vi "Confocal.vi"() -> ()   [LabVIEW 2024]
panel:
  out "appended array":dbl[](array[numeric])
  in  "N per point":i32=1
  in  "Z Steps?":i32
  out "Intensity Graph":dbl[][](graph)
  in  "Direction":bool
  in  "file path (use dialog) 2":path=path "C:/Users/Crawford Group/Desktop/Angelo/NMR/DATA/Unaveraged&TimeStamp.txt"
  in  "file path (use dialog)":path=path "C:/Users/Crawford Group/Desktop/Angelo/NMR/DATA/DATA.txt"
  out "error out":errorcluster
  in  "Step size mm  Y":dbl=0.0017
  in  "Y Motor":refnum<k7>(container)
  out "error out 2":errorcluster
  in  "Step size mm X":dbl=0.0098
  in  "X Motor":refnum<k7>(container)
  in  "Sweeps (X,Y)":i32=1
  in  "Up?":bool
  in  "Number of X steps":dbl=1.0
  out "Number of X":i32
  out "Y Steps":i32
  out "Direction Indicator":bool
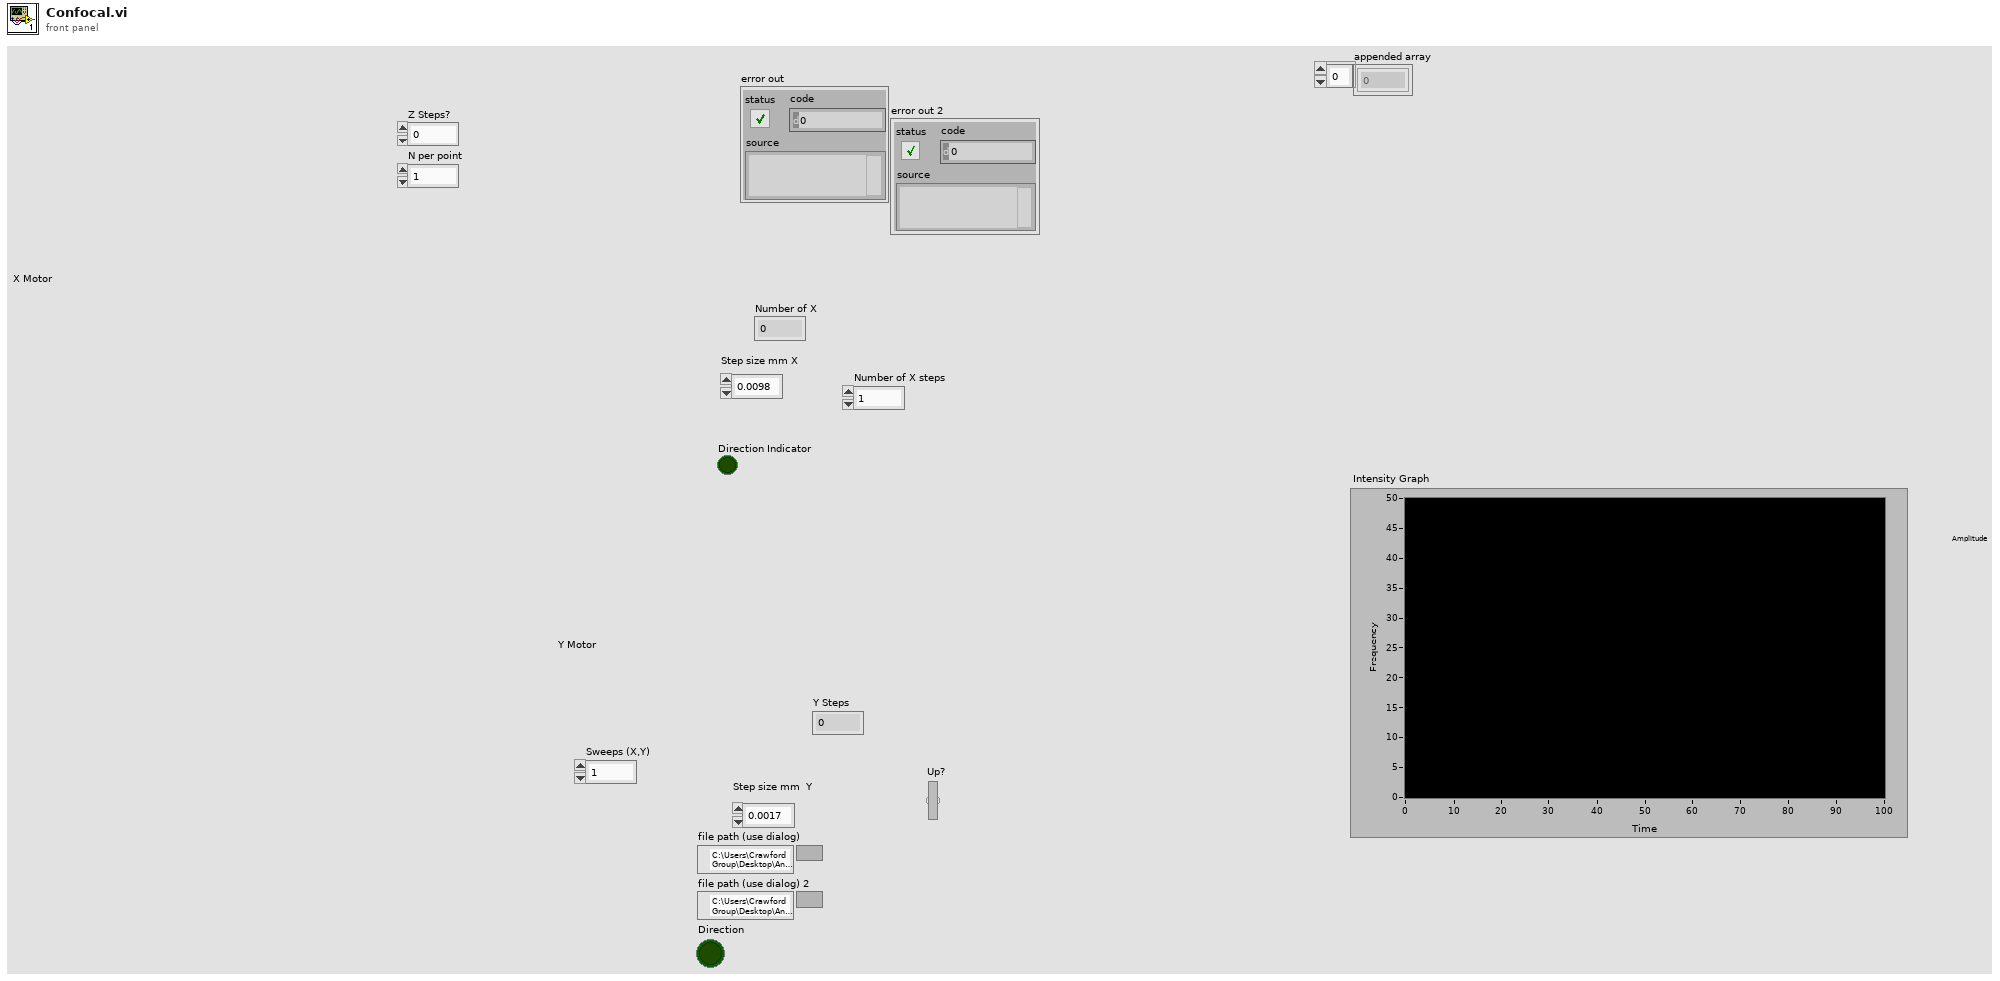
[diagram p1: front panel]
types:
  T1 = enum16{"open", "replace", "create", "open or create", "replace or create", "replace or create with confirmation"}
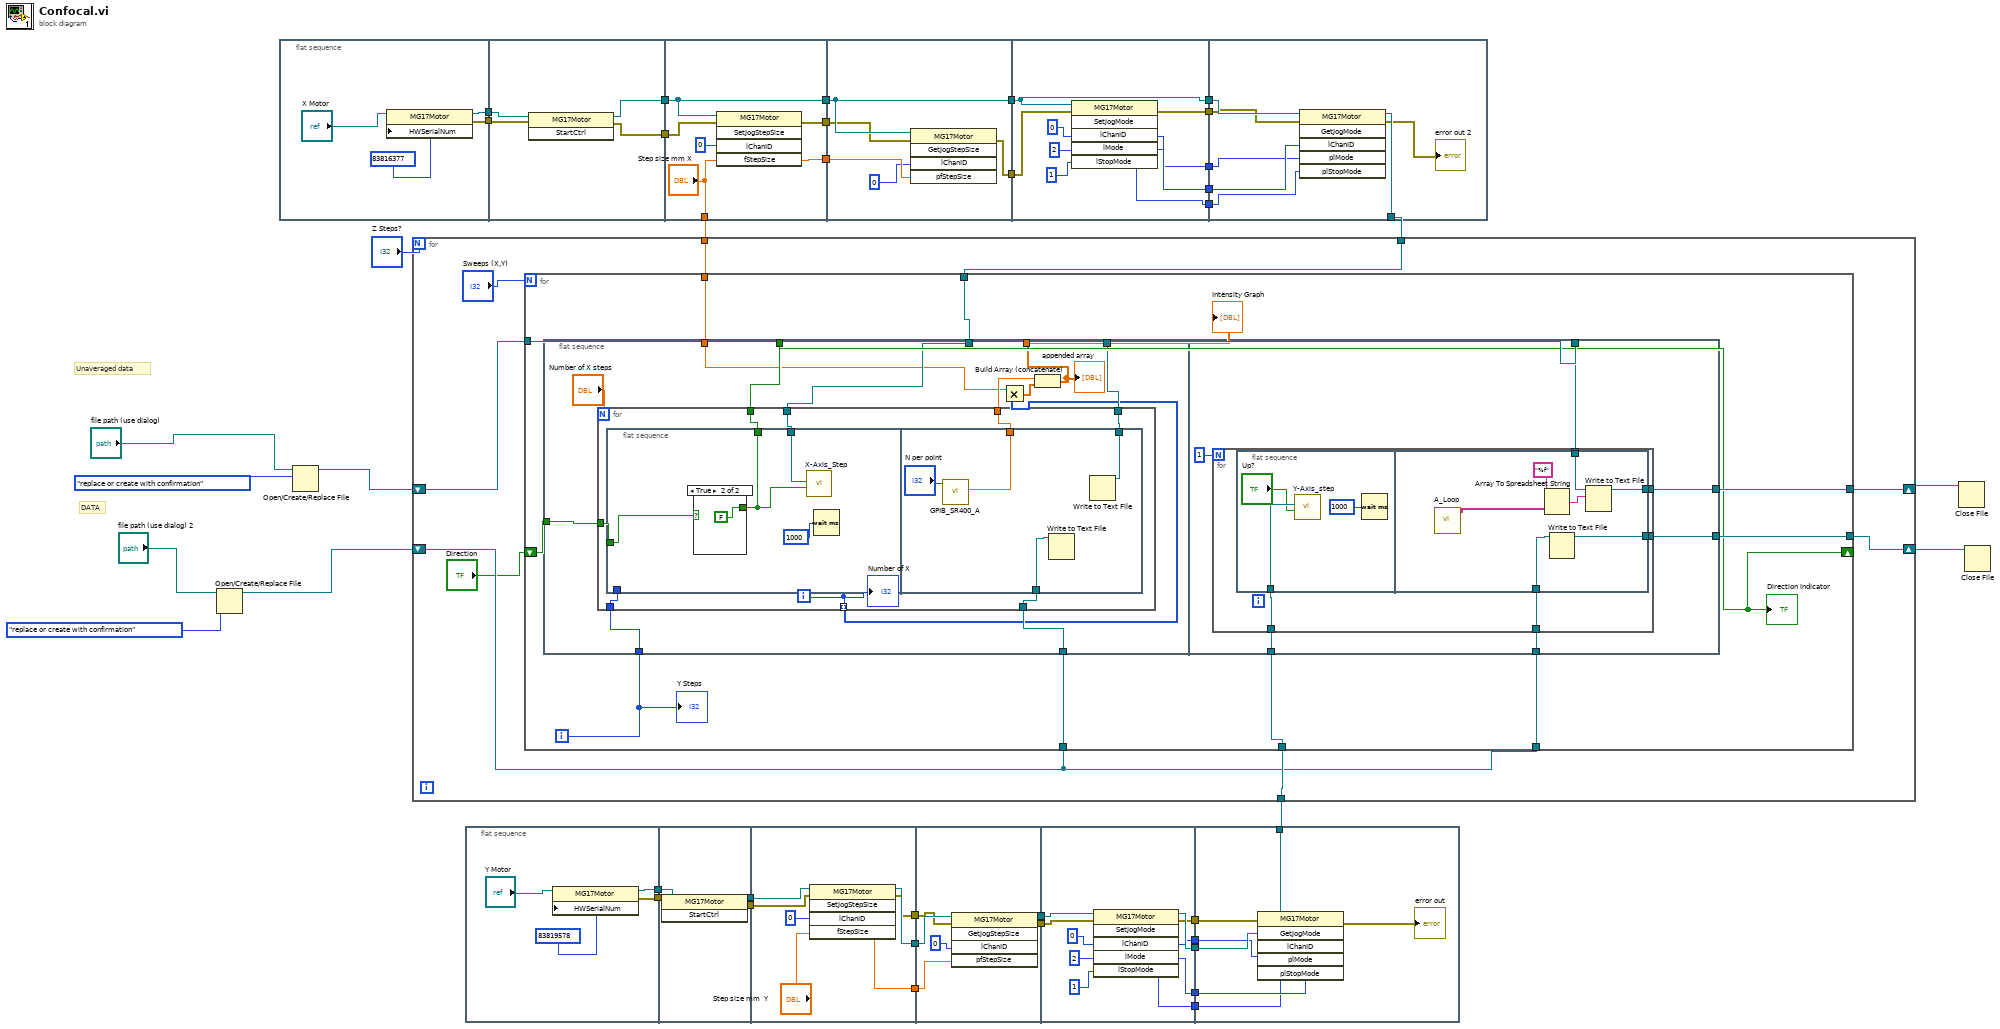
[diagram p0: block diagram]
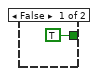
[diagram p2: hidden frame]
diagram:
  # "Unaveraged data"
  # "DATA"
  n1 = Open/Create/Replace File(file path (use dialog)="file path (use dialog) 2", operation (0:open)=T1."replace or create with confirmation") -> (refnum out=w3:refnum<file>)  [unwired: 4 in, 2 out]
  n2 = flat-sequence {
    tunnel: [w42] -> w40
    tunnel: [w41] -> w39
    tunnel: w40 -> [w48]
    tunnel: w39 -> [w47]
    tunnel: [w46] -> w38
    tunnel: [w45] -> w37
    tunnel: w38 -> [w54]
    tunnel: w37 -> [w53]
    tunnel: [w54] -> w36
    tunnel: [w52] -> w35
    tunnel: [w51] -> w34
    tunnel: ["Step size mm X"] -> w1
    tunnel: w36 -> [w59]
    tunnel: w35 -> [w58]
    tunnel: w34 -> [w57]
    tunnel: [w59] -> w33
    tunnel: [w56] -> w32
    tunnel: w33 -> [w68]
    tunnel: w32 -> [w67]
    tunnel: [w68] -> w31
    tunnel: [w63] -> w30
    tunnel: [w62] -> w29
    tunnel: [w61] -> w28
    tunnel: [w60] -> w27
    tunnel: w31 -> [w75]
    tunnel: w30 -> [w74]
    tunnel: w29 -> [w73]
    tunnel: w28 -> [w72]
    tunnel: [w71] -> w12
    tunnel: w27 -> [w69]
    frame #0 {
      n3 = property class="MG17Motor"(reference="X Motor", "HWSerialNum"=83816377) -> (reference out=w42:refnum<k7>, error out=w41:errorcluster)  [unwired: 1 in]
    }
    frame #1 {
      n4 = invoke class="MG17Motor" method="StartCtrl"(reference=w48, error in=w47) -> (reference out=w46:refnum<k7>, error out=w45:errorcluster)  [unwired: 1 in, 1 out]
    }
    frame #2 {
      n5 = invoke class="MG17Motor" method="SetJogStepSize"(reference=w54, error in=w53, "lChanID"=0, "fStepSize"="Step size mm X") -> (error out=w52:errorcluster, "fStepSize"=w51:sgl)  [unwired: 1 in, 3 out]
    }
    frame #3 {
      n6 = invoke class="MG17Motor" method="GetJogStepSize"(reference=w59, error in=w58, "lChanID"=0, "pfStepSize"=w57) -> (error out=w56:errorcluster)  [unwired: 1 in, 4 out]
    }
    frame #4 {
      n7 = invoke class="MG17Motor" method="SetJogMode"(reference=w68, error in=w67, "lChanID"=0, "lMode"=2, "lStopMode"=1) -> (error out=w63:errorcluster, "lChanID"=w62:i32, "lMode"=w61:i32, "lStopMode"=w60:i32)  [unwired: 1 in, 2 out]
    }
    frame #5 {
      n8 = invoke class="MG17Motor" method="GetJogMode"(reference=w75, error in=w74, "lChanID"=w73, "plMode"=w72, "plStopMode"=w69) -> (reference out=w71:refnum<k7>, error out=→"error out 2":errorcluster)  [unwired: 1 in, 4 out]
    }
  }
  n9 = Open/Create/Replace File(file path (use dialog)="file path (use dialog)", operation (0:open)=T1."replace or create with confirmation") -> (refnum out=w5:refnum<file>)  [unwired: 4 in, 2 out]
  n10 = for {
    N: "Z Steps?" -> [_]
    tunnel: w12 -> [w83]
    tunnel: w11 -> [w82]
    shift-right: [w81] -> w6
    shift-left: w5 -> [w80]
    shift-right: [w79] -> w4
    shift-left: w3 -> [w78]
    tunnel: w1 -> [w76]
    n11 = for {
      N: "Sweeps (X,Y)" -> [_]
      tunnel: w82 -> [w96]
      tunnel: w83 -> [w95]
      tunnel: [w94] -> w81
      tunnel: w80 -> [w91]
      tunnel: w78 -> [w93]
      tunnel: [w92] -> w79
      tunnel: w78 -> [w90]
      shift-right: [w87] -> _
      shift-left: "Direction" -> [w88]
      tunnel: w76 -> [w86]
      i -> [w89]
      n12 = flat-sequence {
        tunnel: w95 -> [w100]
        tunnel: w91 -> [w107]
        tunnel: w90 -> [w106]
        tunnel: w89 -> [w105]
        tunnel: w88 -> [w104]
        tunnel: [w103] -> w87
        tunnel: [w101] -> w85
        tunnel: w86 -> [w97]
        tunnel: w96 -> [w132]
        tunnel: [w131] -> w94
        tunnel: w91 -> [w130]
        tunnel: w93 -> [w129]
        tunnel: [w128] -> w92
        frame #0 {
          n13 = for {
            N: "Number of X steps" -> [_]
            tunnel: w107 -> [w116]
            tunnel: w106 -> [w115]
            tunnel: w105 -> [w114]
            tunnel: w104 -> [w113]
            tunnel: [w112] -> w103
            tunnel: [w111] -> w102
            tunnel: w100 -> [w110]
            tunnel: [w109] -> w98 mode=indexing
            i -> [w109]
            n14 = flat-sequence {
              tunnel: w110 -> [w119]
              tunnel: w114 -> [_]
              tunnel: w113 -> [w118]
              tunnel: [w117] -> w112
              tunnel: w116 -> [w126]
              tunnel: w115 -> [w125]
              tunnel: [w123] -> w111
              frame #0 {
                n15 = case shown="True" w118 {
                  tunnel: [TRUE ("Left?") FALSE ("Left?")] -> w117
                  frame False {
                  }
                  frame True {
                  }
                }
                n16 = call "X-Axis_Step.vi"("Left?"=w117, "X Motor"=w119) -> ()  [unwired: 10 in]
                n17 = Wait (ms)(milliseconds to wait=u32 1000) -> ()  [unwired: 1 out]
              }
              frame #1 {
                n18 = call "GPIB_SR400_A.vi"("N per point"="N per point") -> ("x/y"=w123:dbl)  [unwired: 9 in, 1 out]
                n19 = Write to Text File(file (use dialog)=w125) -> ()  [unwired: 3 in, 3 out]
                n20 = Write to Text File(file (use dialog)=w126) -> ()  [unwired: 3 in, 3 out]
              }
            }
            "Number of X" <- w109
          }
          n21 = Multiply(x=w97, y=w98) -> (x*y=w99:dbl[])
          n22 = Build Array (concatenate)(w102, w99) -> (w101:dbl[])
          "appended array" <- w101
        }
        frame #1 {
          n23 = for {
            N: 1 -> [_]
            tunnel: w132 -> [w137]
            tunnel: [w136] -> w131
            tunnel: w130 -> [w135]
            tunnel: w129 -> [w134]
            tunnel: [w133] -> w128
            n24 = flat-sequence {
              tunnel: w137 -> [w139]
              tunnel: [w145] -> w136
              tunnel: w135 -> [w144]
              tunnel: w134 -> [w143]
              tunnel: [w142] -> w133
              frame #0 {
                n25 = call "Y-Axis_step.vi"("Up?"="Up?", "Y Motor"=w139) -> ()  [unwired: 9 in, 1 out]
                n26 = Wait (ms)(milliseconds to wait=u32 1000) -> ()  [unwired: 1 out]
              }
              frame #1 {
                n27 = call "A_Loop.vi"() -> ("Averaged"=w141:string[])  [unwired: 7 in, 4 out]
                n28 = Array To Spreadsheet String(array=w141, 3:"%f" ("format string")) -> (spreadsheet string=w147:string)  [unwired: 1 in]
                n29 = Write to Text File(file (use dialog)=w143) -> (refnum out=w142:refnum<file>)  [unwired: 3 in, 2 out]
                n30 = Write to Text File(file (use dialog)=w144, text=w147) -> (refnum out=w145:refnum<file>)  [unwired: 2 in, 2 out]
              }
            }
          }
        }
      }
      "Y Steps" <- w89
      "Direction Indicator" <- w87
      "Intensity Graph" <- w85
    }
  }
  n31 = flat-sequence {
    tunnel: [w149] -> w26
    tunnel: [w148] -> w25
    tunnel: w26 -> [w155]
    tunnel: w25 -> [w154]
    tunnel: [w153] -> w24
    tunnel: [w152] -> w23
    tunnel: w24 -> [w161]
    tunnel: w23 -> [w160]
    tunnel: [w158] -> w22
    tunnel: [w157] -> w21
    tunnel: [w156] -> w20
    tunnel: w22 -> [w168]
    tunnel: w21 -> [w167]
    tunnel: w20 -> [w165]
    tunnel: [w164] -> w19
    tunnel: [w163] -> w18
    tunnel: w19 -> [w178]
    tunnel: w18 -> [w177]
    tunnel: [w173] -> w17
    tunnel: [w172] -> w16
    tunnel: [w171] -> w15
    tunnel: [w170] -> w14
    tunnel: [w169] -> w13
    tunnel: w17 -> [w184]
    tunnel: w16 -> [w183]
    tunnel: w15 -> [w182]
    tunnel: w14 -> [w181]
    tunnel: w13 -> [w180]
    tunnel: [w179] -> w11
    frame #0 {
      n32 = property class="MG17Motor"(reference="Y Motor", "HWSerialNum"=83819578) -> (reference out=w149:refnum<k7>, error out=w148:errorcluster)  [unwired: 1 in]
    }
    frame #1 {
      n33 = invoke class="MG17Motor" method="StartCtrl"(reference=w155, error in=w154) -> (reference out=w153:refnum<k7>, error out=w152:errorcluster)  [unwired: 1 in, 1 out]
    }
    frame #2 {
      n34 = invoke class="MG17Motor" method="SetJogStepSize"(reference=w161, error in=w160, "lChanID"=0, "fStepSize"="Step size mm  Y") -> (reference out=w158:refnum<k7>, error out=w157:errorcluster, "fStepSize"=w156:sgl)  [unwired: 1 in, 2 out]
    }
    frame #3 {
      n35 = invoke class="MG17Motor" method="GetJogStepSize"(reference=w168, error in=w167, "lChanID"=0, "pfStepSize"=w165) -> (reference out=w164:refnum<k7>, error out=w163:errorcluster)  [unwired: 1 in, 3 out]
    }
    frame #4 {
      n36 = invoke class="MG17Motor" method="SetJogMode"(reference=w178, error in=w177, "lChanID"=0, "lMode"=2, "lStopMode"=1) -> (reference out=w173:refnum<k7>, error out=w172:errorcluster, "lChanID"=w171:i32, "lMode"=w170:i32, "lStopMode"=w169:i32)  [unwired: 1 in, 1 out]
    }
    frame #5 {
      n37 = invoke class="MG17Motor" method="GetJogMode"(reference=w184, error in=w183, "lChanID"=w182, "plMode"=w181, "plStopMode"=w180) -> (reference out=w179:refnum<k7>, error out=→"error out":errorcluster)  [unwired: 1 in, 4 out]
    }
  }
  n38 = Close File(refnum=w6) -> ()  [unwired: 1 in, 2 out]
  n39 = Close File(refnum=w4) -> ()  [unwired: 1 in, 2 out]
